vi "DAQmx.Write.vi"(8 "error in (no error)":errorcluster, 10 "AOwfm":waveform(dbl)[](array[waveform]), 11 "DAQmx in":refnum<class "DAQmx.lvclass">) -> (0 "error out":errorcluster, 3 "DAQmx out":refnum<class "DAQmx.lvclass">, 4 "AO time (s)":dbl=53.0 format="%#_6p")   [LabVIEW 2019, in "DAQmx.lvclass"]
uses:
  DAQmx.lvclass
  DAQmx.lvclass/DAQmx.ctl
  <vilib>/DAQmx/write.llb/DAQmx Write (Analog 1D Wfm NChan NSamp).vi
  <vilib>/DAQmx/miscellaneous.llb/DAQmx Fill In Error Info.vi
  <resource>/objmgr/daqmx.rc
panel:
  out "Number of Samples written per channel":u32[](array[numeric])
  out "Parity Check":bool[](array[boolean])
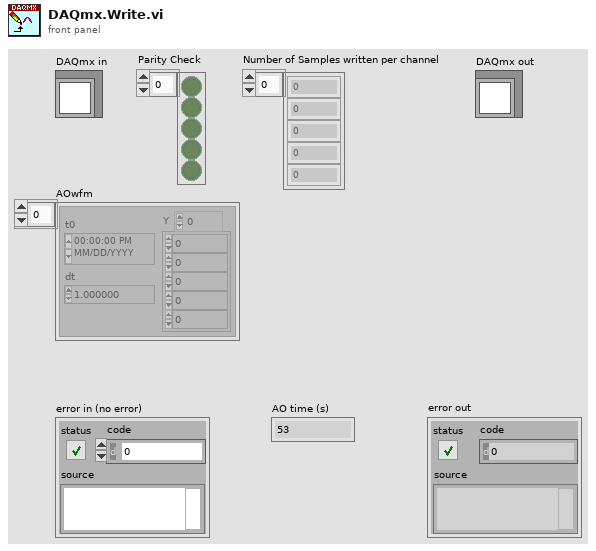
[diagram p1: front panel]
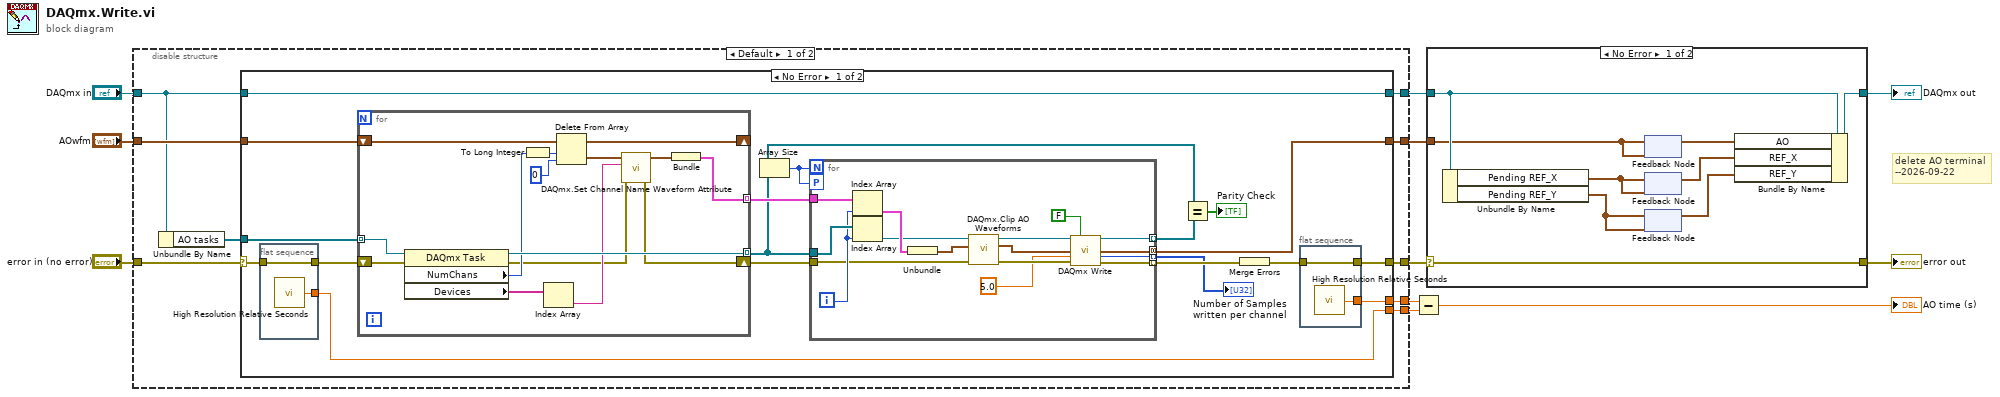
[diagram p0: block diagram]
diagram:
  # "delete AO terminal\n--2026-09-22"
  n1 = disable-structure shown="Default" {
    disable-tunnel: [w20 w76] -> w1
    disable-tunnel: "DAQmx in" -> [w18 w75]
    disable-tunnel: "AOwfm" -> [w19 _]
    disable-tunnel: "error in (no error)" -> [w13 w76]
    disable-tunnel: [w17 w75] -> w4
    disable-tunnel: [w16 _] -> w11
    disable-tunnel: [w15 _] -> w8
    disable-tunnel: [w12 _] -> w5
    frame condition #0 (active) {
      n2 = Unbundle By Name(w18) -> ("AO tasks"=w14:refnum<k21>[])
      n3 = case shown="No Error" w13 {
        selector: w13 -> [w34 w73]
        tunnel: [w36 w73] -> w20
        tunnel: w19 -> [w25 _]
        tunnel: w14 -> [w38 _]
        tunnel: w18 -> [w21 w74]
        tunnel: [w21 w74] -> w17
        tunnel: [w35 _] -> w16
        tunnel: [w32 _] -> w15
        tunnel: [w23 _] -> w12
        frame No Error {
          n4 = flat-sequence {
            tunnel: w34 -> [w41]
            tunnel: [w41] -> w33
            tunnel: [w42] -> w32
            frame #0 {
              n5 = call <vilib>:"High Resolution Relative Seconds.vi"() -> ("relative seconds"=w42:dbl)
            }
          }
          n6 = for {
            tunnel: [w44] -> w30 mode=indexing
            shift-right: [w46] -> w31
            shift-left: w33 -> [w54]
            tunnel: w38 -> [w55] mode=indexing
            shift-right: [w57] -> _
            shift-left: w25 -> [w56]
            tunnel: [w53] -> w24 mode=indexing
            n7 = property class="DAQmx Task"(reference=w55, error in=w54) -> (reference out=w53:refnum<k21>, error out=w45:errorcluster, "NumChans"=w51:u32, "Devices"=w48:tag[])
            n8 = To Long Integer(number=w51) -> (32bit integer=w43:i32)
            n9 = Index Array(array=w48) -> (element=w47:tag)  [unwired: 1 in]
            n10 = Delete From Array(array=w56, length=w43, index=0) -> (deleted portion=w50:waveform(dbl)[], array with subset deleted=w57:waveform(dbl)[])
            n11 = call "DAQmx.Set Channel Name Waveform Attribute.vi"("error in (no error)"=w45, "DAQmx Device Name"=w47, "AOwfm"=w50) -> ("error out"=w46:errorcluster, "Array"=w49:waveform(dbl)[])  [unwired: 7 in]
            n12 = Bundle("Array"=w49) -> (w44:cluster{"Array":waveform(dbl)[]})  [unwired: 1 in]
          }
          n13 = Array Size(array=w24) -> (size(s)=w22:i32)
          n14 = for {
            N: w22 -> [_]
            tunnel: w24 -> [w70]
            tunnel: w30 -> [w71]
            tunnel: w31 -> [w60]
            tunnel: [w68] -> w37 mode=indexing
            workers-P: w22 -> [_]
            tunnel: [w69] -> w28 mode=indexing
            tunnel: [w67] -> w26 mode=indexing
            tunnel: [w61] -> w23 mode=concatenating
            i -> [w65]
            n15 = Index Array(array=w71, index=w65) -> (element=w72:cluster{"Array":waveform(dbl)[]})
            n16 = Index Array(array=w70, index=w65) -> (element=w63:refnum<k21>)
            n17 = Unbundle(w72) -> ("Array"=w64:waveform(dbl)[])
            n18 = call "DAQmx.Clip AO Waveforms.vi"("error in (no error)"=w60, "AO []"=w64, "task"=w63) -> ("error out"=w59:errorcluster, "Clipped AO []"=w61:waveform(dbl)[], "task out"=w62:refnum<k21>)  [unwired: 6 in]
            n19 = call-poly <vilib>:"DAQmx Write.vi"("task/channels in"=w62, "auto start"=FALSE, "data"=w61, "timeout"=5.0, "error in"=w59) -> ("task out"=w69:refnum<k21>, "number of samples written per channel"=w67:u32, "error out"=w68:errorcluster)  [unwired: 8 in]
          }
          "Number of Samples written per channel" <- w26
          n20 = Equal?(x=w24, y=w28) -> (x = y?=→"Parity Check":bool[])
          n21 = Merge Errors(w37) -> (w27:errorcluster)
          n22 = flat-sequence {
            tunnel: w27 -> [w39]
            tunnel: [w39] -> w36
            tunnel: [w40] -> w35
            frame #0 {
              n23 = call <vilib>:"High Resolution Relative Seconds.vi"() -> ("relative seconds"=w40:dbl)
            }
          }
        }
        frame Error {
        }
      }
    }
    frame condition #1 {
    }
  }
  n24 = Subtract(x=w11, y=w8) -> (x-y=→"AO time (s)":dbl)
  n25 = case shown="No Error" w1 {
    selector: w1 -> [w79 w86]
    tunnel: w5 -> [w77 _]
    tunnel: w4 -> [w84 w87]
    tunnel: [w80 w87] -> w3
    tunnel: [w79 w86] -> w2
    frame No Error {
      n26 = Unbundle By Name(w84) -> ("Pending REF_X"=w85:waveform(dbl)[], "Pending REF_Y"=w78:waveform(dbl)[])
      n27 = feedback #1(w77) -> (w83:waveform(dbl)[])
      n28 = feedback-in #1(w77) -> ()
      n29 = feedback #2(w85) -> (w82:waveform(dbl)[])
      n30 = feedback-in #2(w85) -> ()
      n31 = feedback #3(w78) -> (w81:waveform(dbl)[])
      n32 = feedback-in #3(w78) -> ()
      n33 = Bundle By Name(cluster=w84, "AO"=w83, "REF_X"=w82, "REF_Y"=w81) -> (w80:refnum<class "DAQmx.lvclass">)
    }
    frame Error {
    }
  }
  "error out" <- w2
  "DAQmx out" <- w3
